vi "Unitary_Test_Open.vi"() -> (0 "Test_passed":bool)   [LabVIEW 2014]
panel:
  in  "Expected Results":T1(array[cluster])=[{"Controls_list"=[{"Name"="intin", "Type"="int", "Min"="-2147483648", "Max"="2147483647", "Precision"="1", "Description"="integer imput"}, {"Name"="stop", "Type"="boolean", "Min"="false", "Max"="true", "Precision"="", "Description"="Stops the Vi"}, {"Name"="booleanin", "Type"="boolean", "Min"="false", "Max"="true", "Precision"="", "Description"="Boolean input"}, {"Name"="stringin", "Type"="string", "Min"="", "Max"="", "Precision"="", "Description"="String input"}, {"Name"="doublein", "Type"="float", "Min"="-Inf", "Max"="Inf", "Precision"="0", "Description"="double input"}, {"Name"="arrayin", "Type"="array", "Min"="Inf", "Max"="-Inf", "Precision"="0", "Description"=""}], "Indicators_list"=[{"Name"="intout", "Type"="int", "Min"="-2147483648", "Max"="2147483647", "Precision"="1", "Description"="integer outputs"}, {"Name"="stringout", "Type"="string", "Min"="", "Max"="", "Precision"="", "Description"="String output"}, {"Name"="booleanout", "Type"="boolean", "Min"="false", "Max"="true", "Precision"="", "Description"="Boolean output"}, {"Name"="doubleout", "Type"="float", "Min"="-Inf", "Max"="Inf", "Precision"="0", "Description"="double output"}, {"Name"="time", "Type"="float", "Min"="-Inf", "Max"="Inf", "Precision"="0", "Description"="time"}, {"Name"="arrayout", "Type"="array", "Min"="Inf", "Max"="-Inf", "Precision"="0", "Description"=""}], "error out"={"status"=FALSE, "code"=0, "source"=""}}]
  out "Numeric":i32
  out "Results":T1(array[cluster])=[{"Controls_list"=[{"Name"="intin", "Type"="int", "Min"="-2147483648", "Max"="2147483647", "Precision"="1", "Description"="integer imput"}, {"Name"="stop", "Type"="boolean", "Min"="false", "Max"="true", "Precision"="", "Description"="Stops the Vi"}, {"Name"="booleanin", "Type"="boolean", "Min"="false", "Max"="true", "Precision"="", "Description"="Boolean input"}, {"Name"="stringin", "Type"="string", "Min"="", "Max"="", "Precision"="", "Description"="String input"}, {"Name"="doublein", "Type"="float", "Min"="-Inf", "Max"="Inf", "Precision"="0", "Description"="double input"}, {"Name"="arrayin", "Type"="array", "Min"="Inf", "Max"="-Inf", "Precision"="0", "Description"=""}], "Indicators_list"=[{"Name"="intout", "Type"="int", "Min"="-2147483648", "Max"="2147483647", "Precision"="1", "Description"="integer outputs"}, {"Name"="stringout", "Type"="string", "Min"="", "Max"="", "Precision"="", "Description"="String output"}, {"Name"="booleanout", "Type"="boolean", "Min"="false", "Max"="true", "Precision"="", "Description"="Boolean output"}, {"Name"="doubleout", "Type"="float", "Min"="-Inf", "Max"="Inf", "Precision"="0", "Description"="double output"}, {"Name"="time", "Type"="float", "Min"="-Inf", "Max"="Inf", "Precision"="0", "Description"="time"}, {"Name"="arrayout", "Type"="array", "Min"="Inf", "Max"="-Inf", "Precision"="0", "Description"=""}], "error out"={"status"=FALSE, "code"=0, "source"=""}}]
  out "Test_OK":bool[](array[boolean])
  out "hidden":errorcluster
  in  "Array of imputs":string[](array[string])=["TestOK"]
  # "Test basic methods with some testing plant"
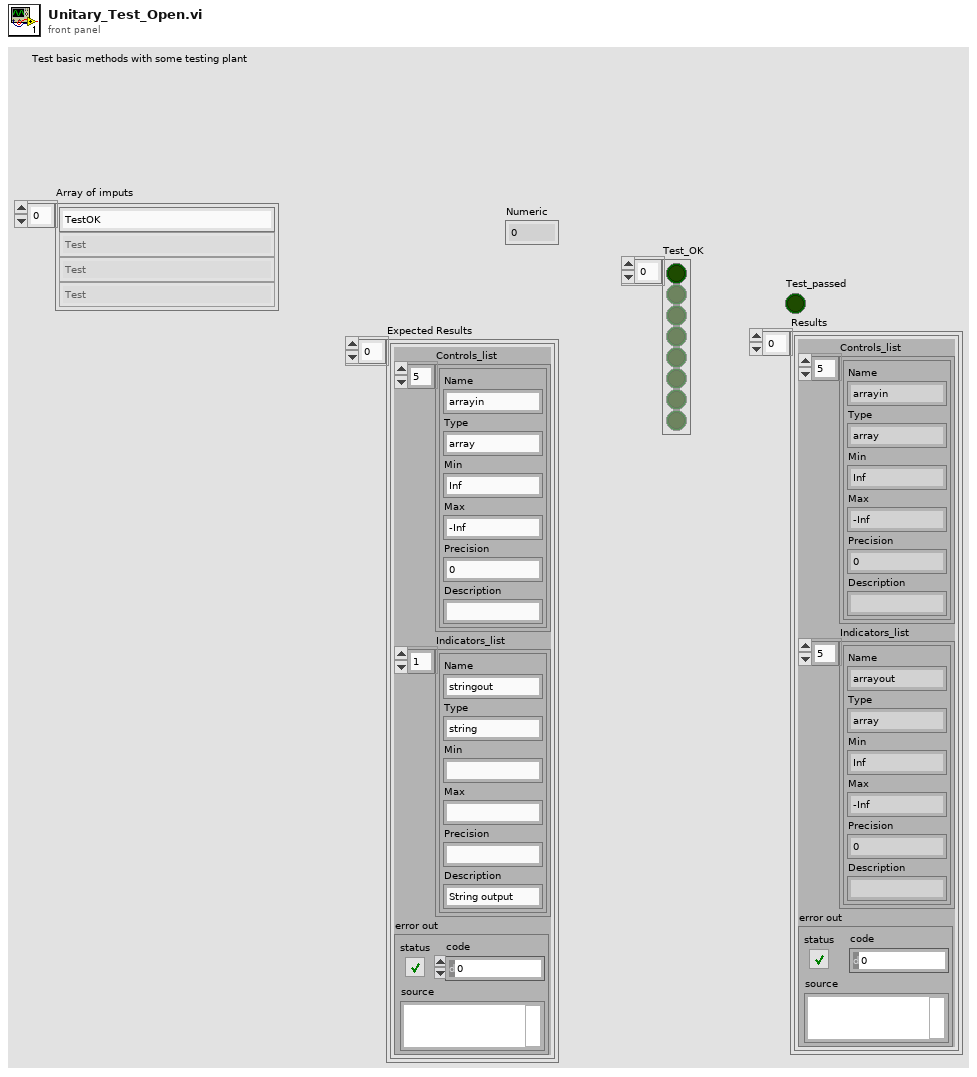
[diagram p1: front panel]
types:
  T1 = cluster{"Controls_list":cluster{"Name":string, "Type":string, "Min":string, "Max":string, "Precision":string, "Description":string}[], "Indicators_list":cluster{"Name":string, "Type":string, "Min":string, "Max":string, "Precision":string, "Description":string}[], "error out":errorcluster}[]
  T2 = cluster{"Name":string, "Type":string, "Min":string, "Max":string, "Precision":string, "Description":string}[]
  T3 = cluster{"Controls_list":cluster{"Name":string, "Type":string, "Min":string, "Max":string, "Precision":string, "Description":string}[], "Indicators_list":cluster{"Name":string, "Type":string, "Min":string, "Max":string, "Precision":string, "Description":string}[], "error out":errorcluster}
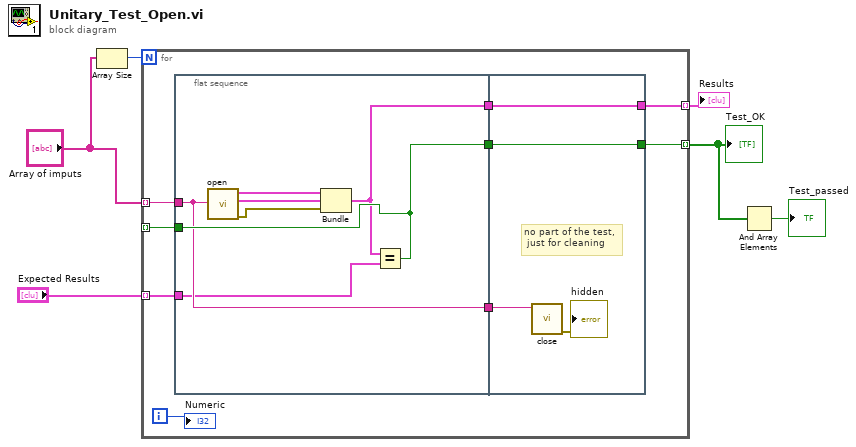
[diagram p0: block diagram]
diagram:
  n1 = Array Size(array="Array of imputs") -> (size(s)=w6:i32)
  n2 = for {
    N: w6 -> [_]
    tunnel: "Array of imputs" -> [w15] mode=indexing
    tunnel: [w13] -> w5 mode=indexing
    tunnel: [w11] -> w3 mode=indexing
    tunnel: [w9] -> _ mode=indexing
    tunnel: "Expected Results" -> [w7] mode=indexing
    i -> [w8]
    n3 = flat-sequence {
      tunnel: w15 -> [w18]
      tunnel: [w18] -> w14
      tunnel: [w19] -> w12
      tunnel: [w16] -> w10
      tunnel: [w19] -> w9
      tunnel: w7 -> [w17]
      tunnel: w14 -> [w26]
      tunnel: [w24] -> w13
      tunnel: w12 -> [w24]
      tunnel: [w23] -> w11
      tunnel: w10 -> [w23]
      frame #0 {
        n4 = call "open.vi"("Experience ID"=w18) -> ("error out"=w20:errorcluster, "Indicators_list"=w21:T2, "Controls_list"=w22:T2)  [unwired: 8 in]
        n5 = Bundle("Controls_list"=w22, "Indicators_list"=w21, "error out"=w20) -> (w16:T3)  [unwired: 1 in]
        n6 = Equal?(x=w16, y=w17) -> (x = y?=w19:bool)
      }
      frame #1 {
        # "no part of the test,\n just for cleaning"
        n7 = call "close.vi"("Experience ID"=w26) -> ("error out"=→"hidden":errorcluster)  [unwired: 10 in]
      }
    }
    "Numeric" <- w8
  }
  "Test_OK" <- w5
  "Results" <- w3
  n8 = And Array Elements(Boolean array=w5) -> (logical AND=→"Test_passed":bool)
